vi "ALL - CalcExpress Toolkit VIs.vi"() -> ()   [LabVIEW 2021]
doc: "::: CalcExpress Toolkit :::\nCopyright (c) 2000-2026 Konstantin Shifershteyn. All rights reserved."
uses:
  cetypes.llb/CalcExpress Instance RefNum.ctl
  cse.llb/CSE Instance RefNum.ctl
  cetypes.llb/VarMan Variable Context Handle.ctl
  cse.llb/CSE Type - Callback Call Reason.ctl
panel:
  in  "False":bool
  # "CalcExpress Toolkit\n\nVI Collection"
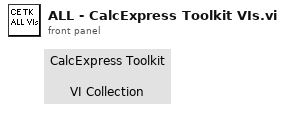
[diagram p1: front panel]
types:
  T1 = typedef "CSE Type - Callback Call Reason.ctl" = u32
  T2 = typedef "VarMan Variable Context Handle.ctl" = i32
  T3 = typedef "CSE Instance RefNum.ctl" = refnum<k1>
  T4 = typedef "CalcExpress Instance RefNum.ctl" = refnum<k1>
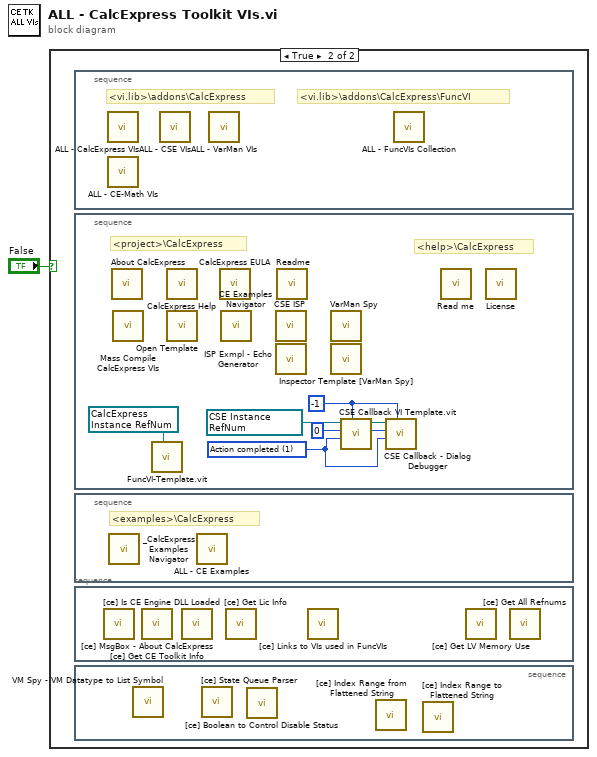
[diagram p0: block diagram]
diagram:
  n1 = case shown="True" "False" {
    frame False {
    }
    frame True {
      n2 = stacked-sequence {
        frame #0 {
          # "<vi.lib>\\addons\\CalcExpress\\FuncVI"
          # "<vi.lib>\\addons\\CalcExpress"
          n3 = call "ALL - CalcExpress VIs.vi"() -> ()  [unwired: 1 in]
          n4 = call "ALL - CE-Math VIs.vi"() -> ()  [unwired: 1 in]
          n5 = call "ALL - CSE VIs.vi"() -> ()  [unwired: 1 in]
          n6 = call "ALL - VarMan VIs.vi"() -> ()  [unwired: 1 in]
          n7 = call "ALL - FuncVIs Collection.vi"() -> ()  [unwired: 1 in]
        }
      }
      n8 = stacked-sequence {
        frame #0 {
          w3 = T1 1 items=["Exec Start", "Action completed", "pause to breath", "reserved 1", "reserved 2", "custom"] ("Call Reason")
          w2 = T2 -1 ("VC Handle")
          w7 = T3 refnum items=["CSE RefNum"] ("CSE RefNum")
          w8 = T4 refnum items=["CE RefNum"] ("InstanceRef")
          # "<help>\\CalcExpress"
          # "<project>\\CalcExpress"
          n9 = call "About CalcExpress.vi"() -> ()  [unwired: 12 in]
          n10 = call "Mass Compile CalcExpress VIs.vi"() -> ()  [unwired: 1 in]
          n11 = call "FuncVI-Template.vit"("InstanceRef"=w8) -> ()  [unwired: 7 in, 2 out]
          n12 = call "CalcExpress Help.vi"() -> ()  [unwired: 12 in]
          n13 = call "Open Template.vi"() -> ()  [unwired: 1 in]
          n14 = call "CalcExpress EULA.vi"() -> ()  [unwired: 12 in]
          n15 = call "CE Examples Navigator.vi"() -> ()  [unwired: 1 in]
          n16 = call "CSE ISP.vi"() -> ()  [unwired: 1 in]
          n17 = call "ISP Exmpl - Echo Generator.vi"() -> ()  [unwired: 1 in]
          n18 = call "Readme.vi"() -> ()  [unwired: 12 in]
          n19 = call "VarMan Spy.vi"() -> ()  [unwired: 1 in]
          n20 = call "Inspector Template [VarMan Spy].vi"() -> ()  [unwired: 1 in]
          n21 = call "CSE Callback VI Template.vit"("VC Handle"=w2, "Call Reason"=w3, "Stm Index"=0, "CSE RefNum"=w7) -> ("Stm Index out"=w4:i32, "dup CSE RefNum"=w5:T3)  [unwired: 2 in, 4 out]
          n22 = call "CSE Callback - Dialog Debugger.vi"("VC Handle"=w2, "Call Reason"=w3, "Stm Index"=w4, "CSE RefNum"=w5) -> ()  [unwired: 2 in, 6 out]
          n23 = call "Read me.vi"() -> ()  [unwired: 12 in]
          n24 = call "License.vi"() -> ()  [unwired: 12 in]
        }
      }
      n25 = stacked-sequence {
        frame #0 {
          # "<examples>\\CalcExpress"
          n26 = call "_CalcExpress Examples Navigator.vi"() -> ()  [unwired: 1 in]
          n27 = call "ALL - CE Examples.vi"() -> ()  [unwired: 12 in]
        }
      }
      n28 = stacked-sequence {
        frame #0 {
          n29 = call "[ce] Is CE Engine DLL Loaded.vi"() -> ()  [unwired: 10 in, 2 out]
          n30 = call "[ce] Get CE Toolkit Info.vi"() -> ()  [unwired: 4 in, 8 out]
          n31 = call "[ce] MsgBox - About CalcExpress.vi"() -> ()  [unwired: 11 in, 1 out]
          n32 = call "[ce] Get Lic Info.vi"() -> ()  [unwired: 10 in, 2 out]
          n33 = call "[ce] Links to VIs used in FuncVIs.vi"() -> ()  [unwired: 1 in]
          n34 = call "[ce] Get LV Memory Use.vi"() -> ()  [unwired: 10 in, 2 out]
          n35 = call "[ce] Get All Refnums.vi"() -> ()  [unwired: 7 in, 5 out]
        }
      }
      n36 = stacked-sequence {
        frame #0 {
          n37 = call "VM Spy - VM Datatype to List Symbol.vi"() -> ()  [unwired: 11 in, 1 out]
          n38 = call "[ce] State Queue Parser.vi"() -> ()  [unwired: 7 in, 3 out]
          n39 = call "[ce] Boolean to Control Disable Status.vi"() -> ()  [unwired: 4 in, 2 out]
          n40 = call "[ce] Index Range from Flattened String.vi"() -> ()  [unwired: 11 in, 1 out]
          n41 = call "[ce] Index Range to Flattened String.vi"() -> ()  [unwired: 11 in, 1 out]
        }
      }
    }
  }
